vi "Single Axis motor_Y(SubVI).vi"(0 "State=1, I":dbl, 1 "Motor=0, I":i32, 2 "Position=0, I":dbl, 3 "User Input":dbl, 4 "Motor Input":dbl, 5 "Backward":bool, 6 "Forward":bool, 7 "Step diff":dbl, 9 "Motor input_L":refnum<vi>, 11 "User input_L":refnum<vi>, 13 "Step diff_L":refnum<vi>) -> (15 "right":bool, 17 "down":bool, 18 "State Chart":i32(graph), 19 "Motor State":dbl, 20 "State=1, O":dbl, 21 "Motor=0, O":i32, 22 "Position=0, O":dbl, 23 "Real Output":dbl, 24 "Motor Position":dbl, 25 "up":bool, 26 "left":bool, 27 "Moving":bool)   [LabVIEW 2018]
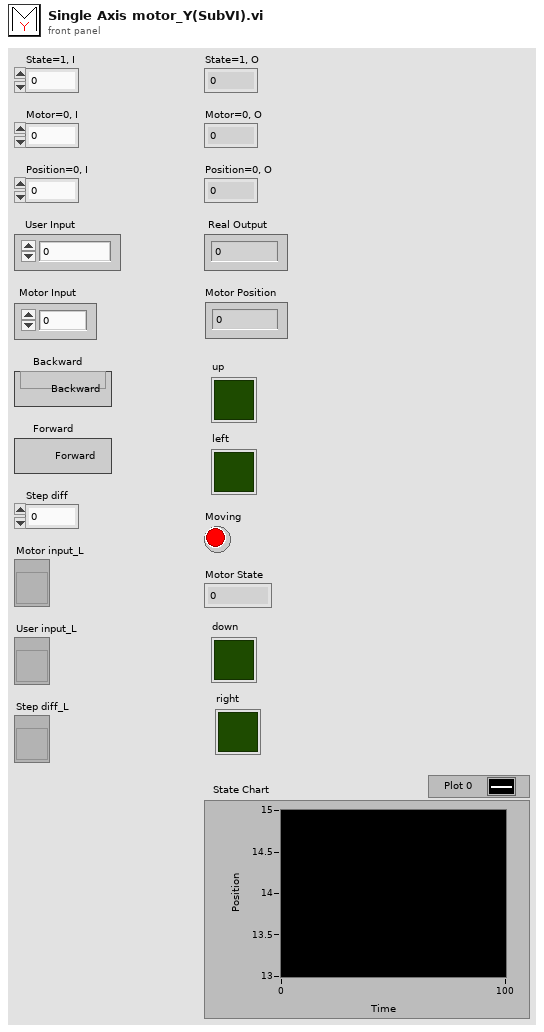
[diagram p1: front panel]
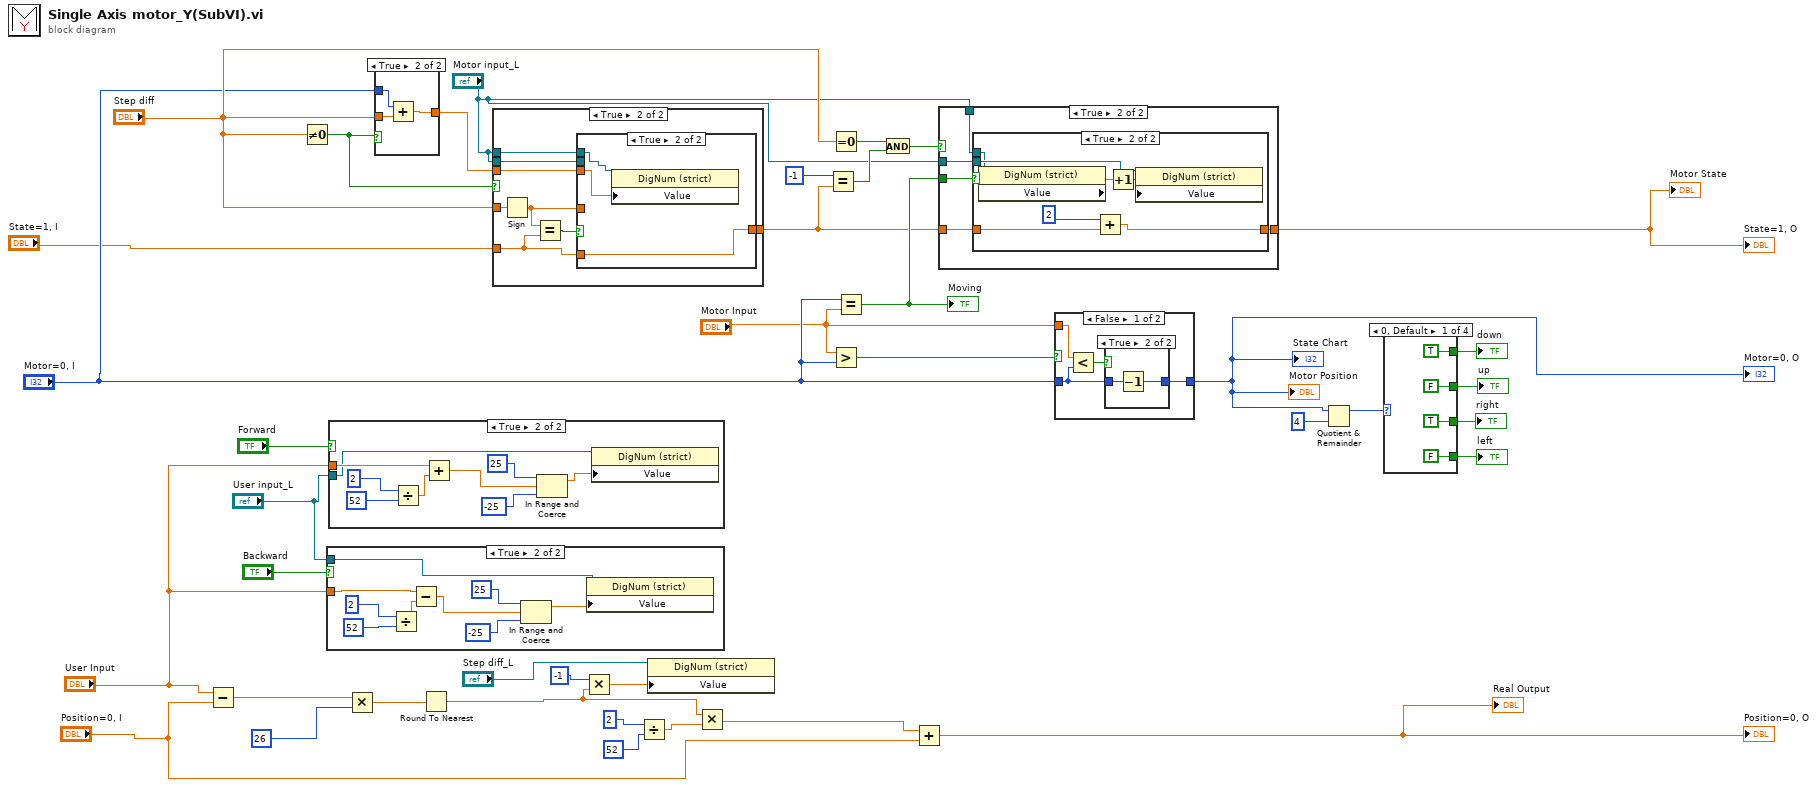
[diagram p0: block diagram]
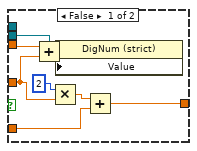
[diagram p7: hidden frame]
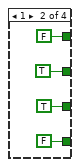
[diagram p8: hidden frame]
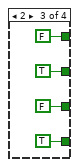
[diagram p9: hidden frame]
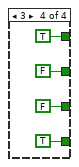
[diagram p10: hidden frame]
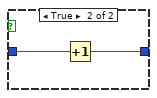
[diagram p12: hidden frame]
diagram:
  n1 = Subtract(x="User Input", y="Position=0, I") -> (x-y=w18:dbl)
  n2 = Not Equal To 0?(x="Step diff") -> (x != 0?=w12:bool)
  n3 = case shown="True" "Backward" {
    tunnel: "User Input" -> [_ w45]
    tunnel: "User input_L" -> [_ w44]
    frame False {
    }
    frame True {
      n4 = Divide(x=2, y=52) -> (x/y=w46:dbl)
      n5 = Subtract(x=w45, y=w46) -> (x-y=w42:dbl)
      n6 = In Range and Coerce(upper limit=25, x=w42, lower limit=-25) -> (coerced(x)=w40:dbl)  [unwired: 1 out]
      n7 = property class="DigNum (strict)"(reference=w44, "Value"=w40) -> ()  [unwired: 1 in, 2 out]
    }
  }
  n8 = case shown="True" "Forward" {
    tunnel: "User Input" -> [_ w54]
    tunnel: "User input_L" -> [_ w53]
    frame False {
    }
    frame True {
      n9 = Divide(x=2, y=52) -> (x/y=w55:dbl)
      n10 = Add(x=w54, y=w55) -> (x+y=w51:dbl)
      n11 = In Range and Coerce(upper limit=25, x=w51, lower limit=-25) -> (coerced(x)=w49:dbl)  [unwired: 1 out]
      n12 = property class="DigNum (strict)"(reference=w53, "Value"=w49) -> ()  [unwired: 1 in, 2 out]
    }
  }
  n13 = Multiply(x=w18, y=26) -> (x*y=w19:dbl)
  n14 = case shown="True" w12 {
    tunnel: "Motor=0, I" -> [_ w61]
    tunnel: "Step diff" -> [w58 w60]
    tunnel: [w58 w59] -> w13
    frame False {
    }
    frame True {
      n15 = Add(x=w61, y=w60) -> (x+y=w59:dbl)
    }
  }
  n16 = Round To Nearest(number=w19) -> (nearest integer value=w2:dbl)
  n17 = case shown="True" w12 {
    tunnel: [w62 w69] -> w28
    tunnel: "State=1, I" -> [w62 w68]
    tunnel: "Step diff" -> [_ w66]
    tunnel: w13 -> [_ w65]
    tunnel: "Motor input_L" -> [_ w64]
    tunnel: "Motor input_L" -> [_ w63]
    frame False {
    }
    frame True {
      n18 = Sign(1:w66) -> (0:w67:dbl)
      n19 = Equal?(x=w67, y=w68) -> (x = y?=w70:bool)
      n20 = case shown="True" w70 {
        tunnel: w67 -> [w72 _]
        tunnel: [w77 w81] -> w69
        tunnel: w68 -> [w75 w81]
        tunnel: w65 -> [w74 w80]
        tunnel: w64 -> [w71 _]
        tunnel: w63 -> [_ w79]
        frame False {
          n21 = Add(x=w74, y=w72) -> (x+y=w76:dbl)
          n22 = Multiply(x=2, y=w72) -> (x*y=w73:dbl)
          n23 = property class="DigNum (strict)"(reference=w71, "Value"=w76) -> ()  [unwired: 1 in, 2 out]
          n24 = Add(x=w73, y=w75) -> (x+y=w77:dbl)
        }
        frame True {
          n25 = property class="DigNum (strict)"(reference=w79, "Value"=w80) -> ()  [unwired: 1 in, 2 out]
        }
      }
    }
  }
  n26 = Multiply(x=-1, y=w2) -> (x*y=w1:dbl)
  n27 = Divide(x=2, y=52) -> (x/y=w22:dbl)
  n28 = property class="DigNum (strict)"(reference="Step diff_L", "Value"=w1) -> ()  [unwired: 1 in, 2 out]
  n29 = Multiply(x=w2, y=w22) -> (x*y=w9:dbl)
  n30 = Equal?(x=-1, y=w28) -> (x = y?=w27:bool)
  n31 = Equal To 0?(x="Step diff") -> (x = 0?=w26:bool)
  n32 = Greater?(x="Motor Input", y="Motor=0, I") -> (0:w11:bool)
  n33 = Equal?(x="Motor=0, I", y="Motor Input") -> (x = y?=w38:bool)
  "Moving" <- w38
  n34 = And(x=w26, y=w27) -> (x .and. y?=w25:bool)
  n35 = Add(x=w9, y="Position=0, I") -> (x+y=→"Real Output" →"Position=0, O":dbl)
  n36 = case shown="True" w25 {
    tunnel: w28 -> [w82 w86]
    tunnel: [w82 w87] -> w24
    tunnel: w38 -> [_ w85]
    tunnel: "Motor input_L" -> [_ w84]
    tunnel: "Motor input_L" -> [_ w83]
    frame False {
    }
    frame True {
      n37 = case shown="True" w85 {
        tunnel: [w88 w93] -> w87
        tunnel: w86 -> [w88 w94]
        tunnel: w84 -> [_ w90]
        tunnel: w83 -> [_ w89]
        frame False {
        }
        frame True {
          n38 = property class="DigNum (strict)"(reference=w89) -> ("Value"=w91:dbl)  [unwired: 1 in, 2 out]
          n39 = Add(x=2, y=w94) -> (x+y=w93:dbl)
          n40 = Increment(x=w91) -> (x+1=w92:dbl)
          n41 = property class="DigNum (strict)"(reference=w90, "Value"=w92) -> ()  [unwired: 1 in, 2 out]
        }
      }
    }
  }
  "Motor State" <- w24
  "State=1, O" <- w24
  n42 = case shown="False" w11 {
    tunnel: "Motor=0, I" -> [w97 w104]
    tunnel: [w96 w103] -> w23
    tunnel: "Motor Input" -> [w99 _]
    frame False {
      n43 = Less?(x=w99, y=w97) -> (x < y?=w98:bool)
      n44 = case shown="True" w98 {
        tunnel: w97 -> [w100 w102]
        tunnel: [w100 w101] -> w96
        frame False {
        }
        frame True {
          n45 = Decrement(x=w102) -> (x-1=w101:i32)
        }
      }
    }
    frame True {
      n46 = Increment(x=w104) -> (x+1=w103:i32)
    }
  }
  "State Chart" <- w23
  "Motor Position" <- w23
  "Motor=0, O" <- w23
  n47 = Quotient & Remainder(x=w23, y=4) -> (x-y*floor(x/y)=w30:i32)  [unwired: 1 out]
  n48 = case shown="0, Default" w30 {
    tunnel: [FALSE FALSE TRUE TRUE] -> w34
    tunnel: [TRUE TRUE FALSE FALSE] -> w33
    tunnel: [FALSE TRUE TRUE FALSE] -> w32
    tunnel: [TRUE FALSE FALSE TRUE] -> w31
    frame 0, Default {
    }
    frame 1 {
    }
    frame 2 {
    }
    frame 3 {
    }
  }
  "up" <- w32
  "down" <- w31
  "right" <- w33
  "left" <- w34
